vi "Room_Images.vi"(0 "Room ID":string="005", 5 "Theme":i32, 11 "error in":errorcluster) -> (4 "Lit":u8[][](array[numeric]), 6 "Dim":u8[][](array[numeric]), 8 "Dark":u8[][](array[numeric]), 10 "Template":T1, 15 "error out":errorcluster)   [LabVIEW 2020, in "GH_Render.lvlib"]
doc: "Loads the three pictures of a room for a colour theme (room_<Theme>_<ID>.png, _dim, _dark) as rasters of 640 rows x 3840 bytes (24 bit). Template = image data of the lit picture without pixels (type, depth, colours)."
uses:
  GH_Render.lvlib
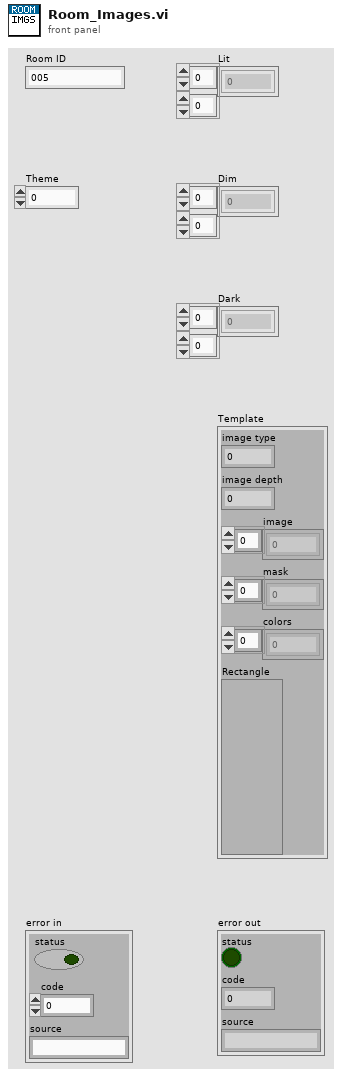
[diagram p1: front panel]
types:
  T1 = cluster{"image type":i32, "image depth":i32, "image":u8[], "mask":u8[], "colors":u32[], "Rectangle":cluster{"left":i16, "top":i16, "right":i16, "bottom":i16}}
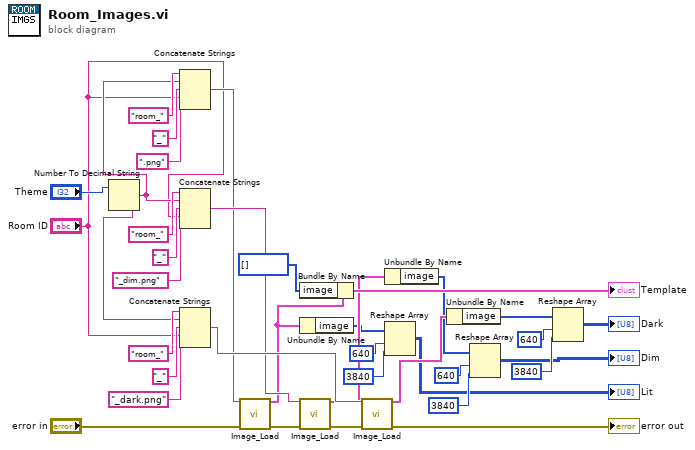
[diagram p0: block diagram]
diagram:
  n1 = Number To Decimal String(number="Theme") -> (decimal integer string=w4:string)  [unwired: 1 in]
  n2 = Concatenate Strings("room_", w4, "_", "Room ID", ".png") -> (w8:string)
  n3 = Concatenate Strings("room_", w4, "_", "Room ID", "_dim.png") -> (w18:string)
  n4 = Concatenate Strings("room_", w4, "_", "Room ID", "_dark.png") -> (w28:string)
  n5 = call "Image_Load.vi"("File name"=w8, "error in"="error in") -> ("Image"=w9:T1, "error out"=w10:errorcluster)  [unwired: 12 in]
  n6 = Bundle By Name(cluster=w9, "image"=u8[] []) -> (→"Template":T1)
  n7 = Unbundle By Name(w9) -> ("image"=w11:u8[])
  n8 = call "Image_Load.vi"("File name"=w18, "error in"=w10) -> ("Image"=w19:T1, "error out"=w20:errorcluster)  [unwired: 12 in]
  n9 = call "Image_Load.vi"("File name"=w28, "error in"=w20) -> ("Image"=w29:T1, "error out"=→"error out":errorcluster)  [unwired: 12 in]
  n10 = Unbundle By Name(w19) -> ("image"=w21:u8[])
  n11 = Reshape Array(w11, 640, 3840) -> (→"Lit":u8[][])
  n12 = Unbundle By Name(w29) -> ("image"=w31:u8[])
  n13 = Reshape Array(w21, 640, 3840) -> (→"Dim":u8[][])
  n14 = Reshape Array(w31, 640, 3840) -> (→"Dark":u8[][])
